vi "Shoot Controller.vi"(8 "error in":errorcluster) -> ()   [LabVIEW 2025]
doc: "This VI executes continuously carrying out the current operation and responding to updates or new operations. It will often contain the timing or control code that is difficult to place directly in TeleOp. This VI generally opens all sensors and motors and isolates the rest of the robot code from knowing how the operations are carried out."
uses:
  <vilib>/Rock Robotics/WPI/Framework/Completion Status.ctl
  <vilib>/Rock Robotics/WPI/ThirdParty/REV Robotics/REVLib/Typedef/SPARK PID Gains.ctl
  <vilib>/Rock Robotics/WPI/ThirdParty/REV Robotics/REVLib/Typedef/SPARK Feed Forward Gains.ctl
  Shoot Setpoints.ctl
  Shoot Operations.ctl
  <vilib>/Rock Robotics/WPI/ThirdParty/REV Robotics/REVLib/Typedef/Spark MAX Control Type.ctl
  79b9af25-1ada-4b96-a7ac-b17063e53c1a.vi
  c9f4092f-8ff2-42f3-87f9-18e20bac81df.vi
  8d211d2e-a7e4-4be3-a004-de462b7f292d.vi
  2d0b4ef1-ddff-4f8f-9f7d-9574eeafe7ac.vi
  <vilib>/Rock Robotics/WPI/ThirdParty/REV Robotics/REVLib/SubVI/Public/SPARK Open Brushless.vi
  <vilib>/Rock Robotics/WPI/ThirdParty/REV Robotics/REVLib/SubVI/Public/SPARK Get Encoder Status Velocity.vi
  <vilib>/Rock Robotics/WPI/ThirdParty/REV Robotics/REVLib/SubVI/Public/SPARK Configure Closed Loop Gains.vi
  <vilib>/Rock Robotics/WPI/ThirdParty/REV Robotics/REVLib/SubVI/Public/SPARK Configure Closed Loop Output Range.vi
  <vilib>/Rock Robotics/Network Tables/NT Write Boolean.vi
panel:
  in  "PID Gains I":T1={"kP"=1e-05, "kI"=0.0, "kD"=0.0}
  in  "Feed Forward Gains I":T2={"kV"=0.003, "kS"=0.0, "kA"=0.0, "kG"=0.0, "kCos"=0.0, "kCosRatio"=0.0}
  in  "Max out Intake":dbl=1.0
  in  "Min out Intake":dbl=-1.0
  out "Intake":T3(graph)
  out "Shooter":T3(graph)
  in  "Intake/Agitater speed":dbl=2500.0
  in  "Shooter Speed":dbl=-5676.0
  in  "Max out Shooter":dbl=1.0
  in  "Min out Shooter":dbl=-1.0
  in  "Feed Forward Gains S":T2={"kV"=0.0021, "kS"=0.0, "kA"=0.0, "kG"=0.0, "kCos"=0.0, "kCosRatio"=0.0}
  in  "PID Gains S":T1={"kP"=0.0001, "kI"=0.0, "kD"=0.0}
  out "Current\nCmd":string="Started at  23:18:34.977\n: Immediate,  S 0.0, D 0.000000"
  in  "Buttons":cluster{"Execute Cmd":bool, "Abort Cmd":bool}
  out "Command Timing":cluster{"Start Time (ms)":u32, "Iterations":i32}
  out "Status":T4
  # "Interactive Command: You may fill in the settings for a command\nand schedule it with the Execute button. You can observe and abort\nany command while fine tuning the code for the controller."
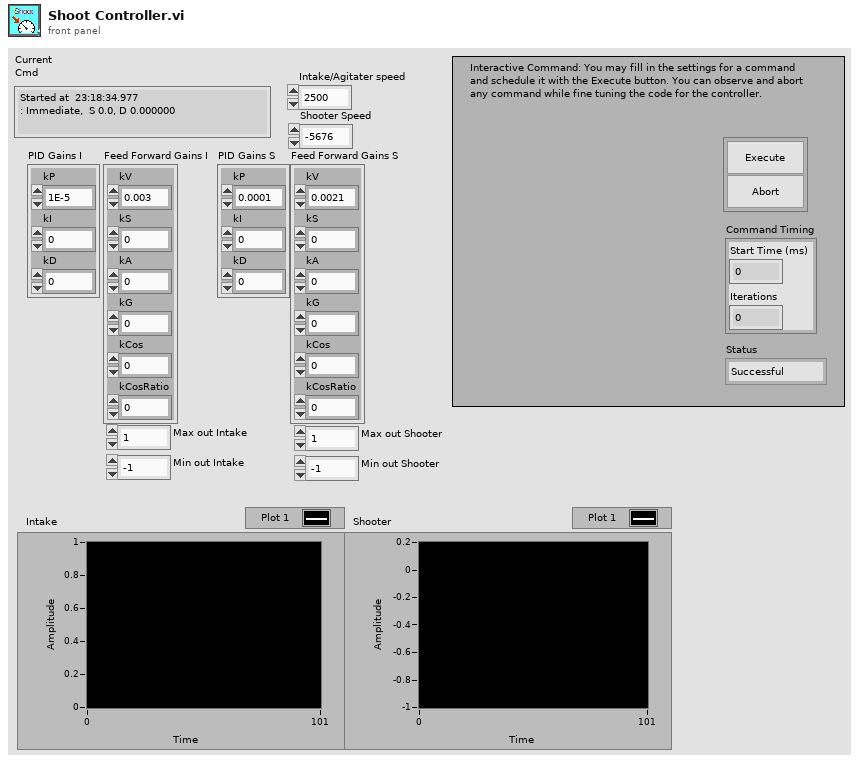
[diagram p1: front panel]
types:
  T1 = typedef "SPARK PID Gains.ctl" = cluster{"kP":dbl, "kI":dbl, "kD":dbl}
  T2 = typedef "SPARK Feed Forward Gains.ctl" = cluster{"kV":dbl, "kS":dbl, "kA":dbl, "kG":dbl, "kCos":dbl, "kCosRatio":dbl}
  T3 = cluster{"Don't move motors while reserved":dbl, "Sensor Velocity":dbl}
  T4 = typedef "Completion Status.ctl" = enum16{"Successful", "Aborted", "Incomplete"}
  T5 = typedef "Shoot Setpoints.ctl" = cluster{"Operation":T6, "Invert Intake":bool, "Shoot":bool, "Intake":bool}
  T6 = typedef "Shoot Operations.ctl" = enum16{"Reserve", "Read Current", "Immediate", "Shoot fuel out the top, intake, and agitate the fuel."}
  T7 = typedef "Command Status Info.ctl" = cluster{"Name":string, "Status":T4, "notifier out":T8}
  T8 = typedef "Completion Notifier.ctl" = refnum<notifier>
  T9 = cluster{"Current Command":T5, "Command Timing":cluster{"Start Time (ms)":u32, "Iterations":i32}, "Command Arguments":cluster{"Command Info":T7, "Description":string, "Default Command":T5, "queue out":refnum<queue>, "Subsystem Name":string}}
  T10 = typedef "WPI_MotorControlDeviceRef.ctl" = cluster{"DeviceStatus":errorcluster, "Type":T11, "PWM":cluster{"PWM Channel":T12, "DeadBand":T13}, "CAN":cluster{"Device Number":u8, "SetOutput VI Ref":variant, "GetOutput VI Ref":variant, "Enable VI Ref":variant, "Disable VI Ref":variant, "Data":variant}, "Invert":bool, "DIO PWM":cluster{"PWM \"Enable\" Channel":T12, "DIOChannel":T14, "PWM Rate":dbl}}
  T11 = typedef "WPI_MotorControlType.ctl" = enum16{"PWM", "CAN", "DIO PWM"}
  T12 = typedef "FPGA_DIOPWMChannel.ctl" = enum8{"PWM 0", "PWM 1", "PWM 2", "PWM 3", "PWM 4", "PWM 5", "PWM 6", "PWM 7", "PWM 8", "PWM 9", "PWM MXP 0", "PWM MXP 1", "PWM MXP 2", "PWM MXP 3", "PWM MXP 4", "PWM MXP 5", "PWM MXP 6", "PWM MXP 7", "PWM MXP 8", "PWM MXP 9", "Invalid"}
  T13 = typedef "WPI_PWMDeadband.ctl" = cluster{"Name":string, "maxPositivePwm":i32, "minPositivePwm":i32, "centerPwm":i32, "maxNegativePwm":i32, "minNegativePwm":i32, "angularRange":u16}
  T14 = typedef "FPGA_DIOChannel.ctl" = enum8{"DIO 0", "DIO 1", "DIO 2", "DIO 3", "DIO 4", "DIO 5", "DIO 6", "DIO 7", "DIO 8", "DIO 9", "DIO MXP 0", "DIO MXP 1", "DIO MXP 2", "DIO MXP 3", "DIO MXP 4", "DIO MXP 5", "DIO MXP 6", "DIO MXP 7", "DIO MXP 8", "DIO MXP 9", "DIO MXP 10", "DIO MXP 11", "DIO MXP 12", "DIO MXP 13", "DIO MXP 14", "DIO MXP 15", "SPI Port CS1", "SPI Port CS2", "SPI Port CS3", "SPI Port MISO", "SPI Port MOSI", "Invalid"}
  T15 = cluster{"Min out Intake":dbl, "Sensor Velocity":dbl}
  T16 = cluster{"Max out Intake":dbl, "Sensor Velocity":dbl}
  T17 = typedef "Spark MAX Control Type.ctl" = enum16{"Percent VBus", "Voltage", "Velocity", "Position", "Smart Motion", "Current", "Smart Velocity", "MAXMotion Position", "MAXMotion Velocity"}
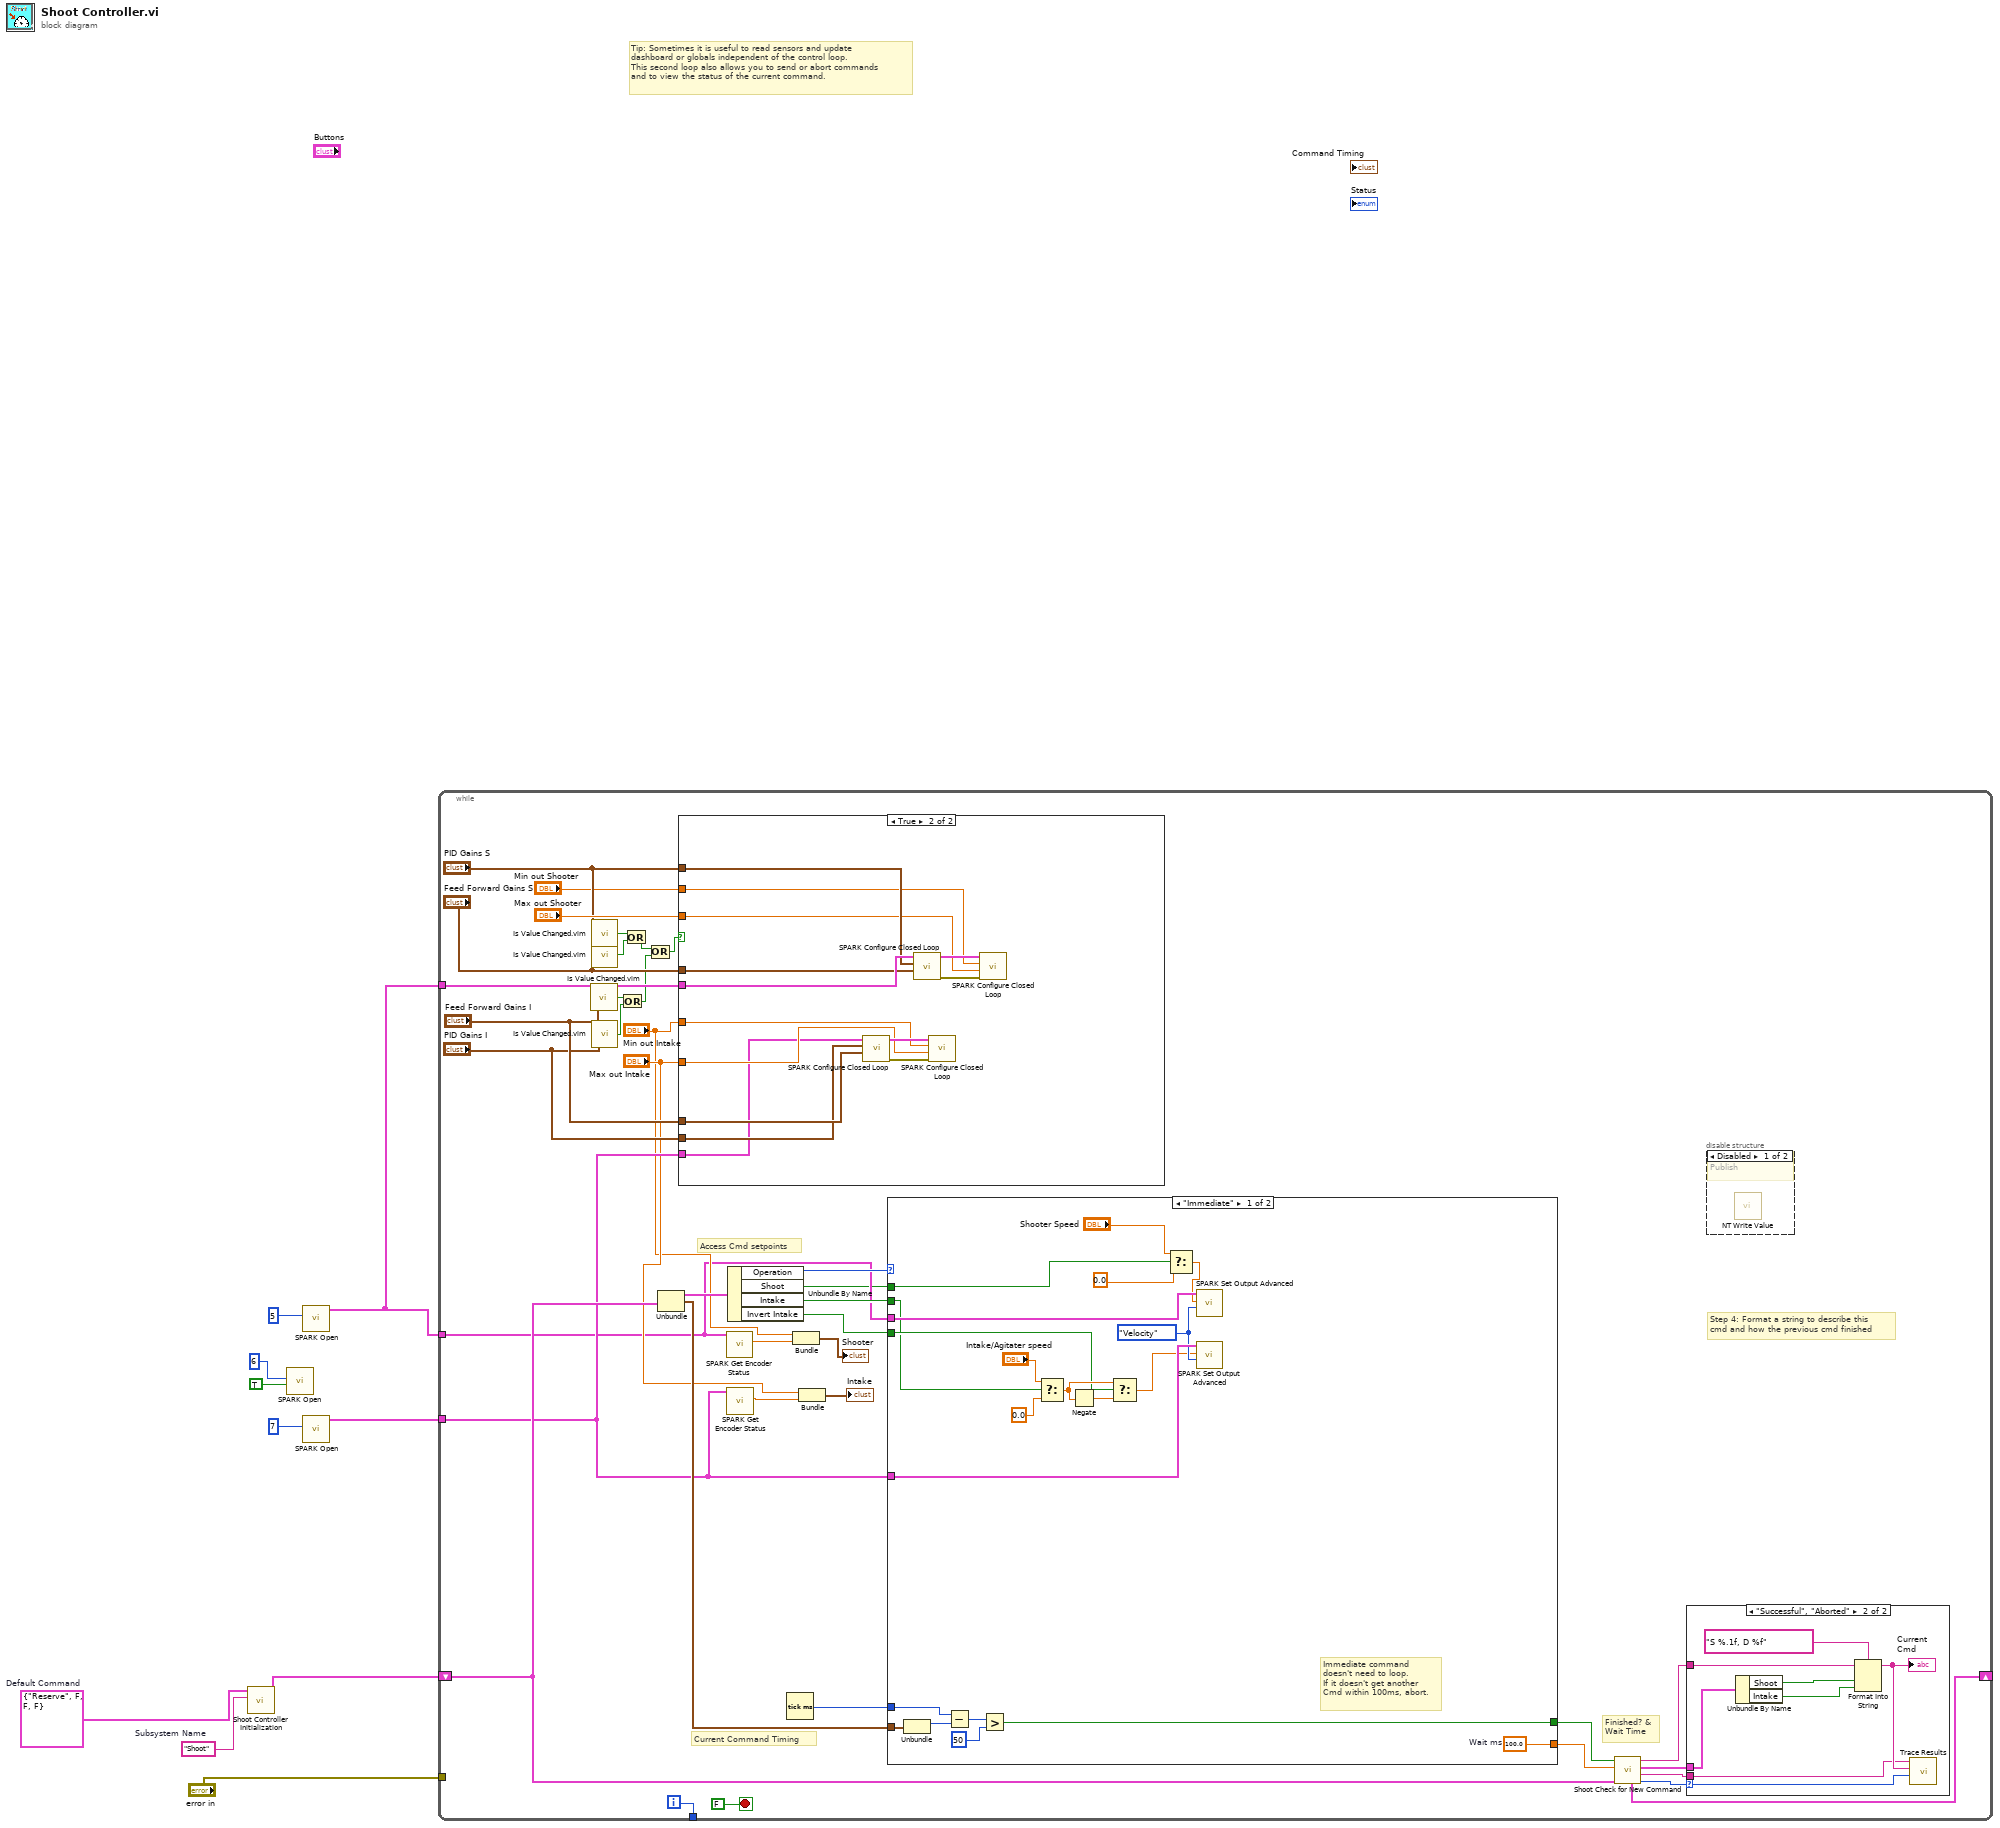
[diagram p0: block diagram]
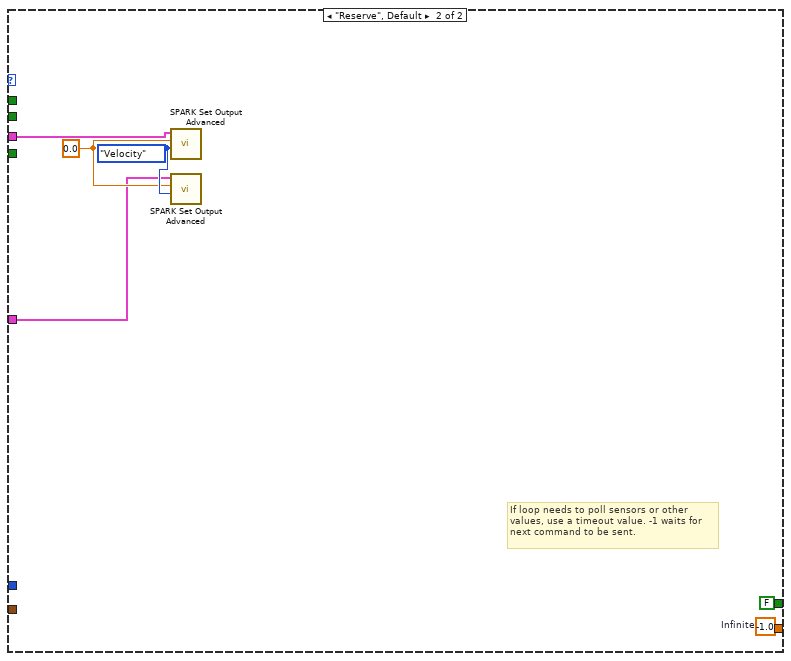
[diagram p5: hidden frame]
diagram:
  w7 = T5 {"Operation"=enum."Reserve", "Invert Intake"=FALSE, "Shoot"=FALSE, "Intake"=FALSE}  # Default Command
  w8 = "Shoot"  # Subsystem Name
  # "Tip: Sometimes it is useful to read sensors and update\ndashboard or globals independent of the control loop.\nThis second loop also allows you to send or abort commands\nand to view the status of the current command."
  n1 = call "Shoot Controller Initialization.vi"("Subsystem Name"=w8, "Default Command"=w7) -> ("Current Command"=w9:T9)  [unwired: 9 in]
  n2 = call-poly <vilib>:"SPARK Open.vi"("Invert"=TRUE, "Device Number"=u8 6) -> ()  [unwired: 8 in, 2 out]
  n3 = call-poly <vilib>:"SPARK Open.vi"("Device Number"=u8 5) -> ("MotorControlDeviceRef"=w1:T10)  [unwired: 9 in, 1 out]
  n4 = call-poly <vilib>:"SPARK Open.vi"("Device Number"=u8 7) -> ("MotorControlDeviceRef"=w3:T10)  [unwired: 9 in, 1 out]
  n5 = while {
    shift-right: [w43] -> _
    shift-left: w9 -> [w36]
    tunnel: [w48] -> _
    tunnel: "error in" -> [_]
    tunnel: w1 -> [w35]
    tunnel: w3 -> [w18]
    tunnel: w1 -> [w13]
    i -> [w48]
    stop <- FALSE stop-if-true
    # "Step 4: Format a string to describe this\ncmd and how the previous cmd finished"
    # "Current Command Timing"
    # "Access Cmd setpoints"
    # "Finished? &\nWait Time"
    n6 = call "Is Value Changed.vim"("value"="Feed Forward Gains I") -> ("changed or first call?"=w24:bool)
    n7 = call "Is Value Changed.vim"("value"="PID Gains S") -> ("changed or first call?"=w34:bool)
    n8 = call "Is Value Changed.vim"("value"="Feed Forward Gains S") -> ("changed or first call?"=w30:bool)
    n9 = call "Is Value Changed.vim"("value"="PID Gains I") -> ("changed or first call?"=w25:bool)
    n10 = Or(x=w24, y=w25) -> (x .or. y?=w26:bool)
    n11 = Or(x=w34, y=w30) -> (x .or. y?=w27:bool)
    n12 = Or(x=w27, y=w26) -> (x .or. y?=w12:bool)
    n13 = Unbundle(w36) -> ("Current Command"=w47:T5, "Command Timing"=w44:cluster{"Start Time (ms)":u32, "Iterations":i32})  [unwired: 1 out]
    n14 = case shown="True" w12 {
      tunnel: w35 -> [_ w63]
      tunnel: "PID Gains S" -> [_ w60]
      tunnel: "Feed Forward Gains S" -> [_ w59]
      tunnel: "Min out Shooter" -> [_ w58]
      tunnel: "Max out Shooter" -> [_ w57]
      tunnel: "Min out Intake" -> [_ w53]
      tunnel: "Max out Intake" -> [_ w54]
      tunnel: "Feed Forward Gains I" -> [_ w52]
      tunnel: "PID Gains I" -> [_ w51]
      tunnel: w18 -> [_ w50]
      frame False {
      }
      frame True {
        n15 = call-poly <vilib>:"SPARK Configure Closed Loop.vi"("Feed Forward Gains"=w52, "PID Gains"=w51, "MotorControlDeviceRef in"=w50) -> ("error out"=w55:errorcluster, "MotorControlDeviceRef out"=w56:T10)  [unwired: 7 in]
        n16 = call-poly <vilib>:"SPARK Configure Closed Loop.vi"("Feed Forward Gains"=w59, "PID Gains"=w60, "MotorControlDeviceRef in"=w63) -> ("error out"=w61:errorcluster, "MotorControlDeviceRef out"=w62:T10)  [unwired: 7 in]
        n17 = call-poly <vilib>:"SPARK Configure Closed Loop.vi"("error in"=w55, "Maximum Output"=w54, "Minimum Output"=w53, "MotorControlDeviceRef in"=w56) -> ()  [unwired: 6 in, 2 out]
        n18 = call-poly <vilib>:"SPARK Configure Closed Loop.vi"("error in"=w61, "Maximum Output"=w57, "Minimum Output"=w58, "MotorControlDeviceRef in"=w62) -> ()  [unwired: 6 in, 2 out]
      }
    }
    n19 = call-poly <vilib>:"SPARK Get Encoder Status.vi"("MotorControlDevRef in"=w13) -> ("Sensor Velocity"=w19:dbl)  [unwired: 7 in, 3 out]
    n20 = call-poly <vilib>:"SPARK Get Encoder Status.vi"("MotorControlDevRef in"=w18) -> ("Sensor Velocity"=w21:dbl)  [unwired: 7 in, 3 out]
    n21 = Unbundle By Name(w47) -> ("Operation"=w46:T6, "Shoot"=w11:bool, "Intake"=w20:bool, "Invert Intake"=w28:bool)
    n22 = Tick Count (ms)() -> (millisecond timer value=w45:u32)
    n23 = Bundle("Min out Intake"="Min out Intake", "Sensor Velocity"=w19) -> (→"Shooter":T15)  [unwired: 1 in]
    n24 = Bundle("Max out Intake"="Max out Intake", "Sensor Velocity"=w21) -> (→"Intake":T16)  [unwired: 1 in]
    n25 = case shown="\"Immediate\"" w46 {
      tunnel: [w92 w98] -> w41
      tunnel: [w86 FALSE ("ignore previous (F)")] -> w42
      tunnel: w44 -> [w88 _]
      tunnel: w11 -> [w72 _]
      tunnel: w45 -> [w87 _]
      tunnel: w20 -> [w73 _]
      tunnel: w13 -> [w85 w96]
      tunnel: w18 -> [w84 w93]
      tunnel: w28 -> [w76 _]
      frame "Immediate" {
        w83 = Spark_MAX_Control_Type."Velocity" ("Control Mode")
        w92 = 100.0  # Wait ms
        # "Immediate command\ndoesn't need to loop.\nIf it doesn't get another\nCmd within 100ms, abort."
        n26 = Unbundle(w88) -> ("Start Time (ms)"=w91:u32)  [unwired: 1 out]
        n27 = Subtract(x=w87, y=w91) -> (x-y=w90:u32)
        n28 = Greater?(x=w90, y=u8 50 ("Left Motor")) -> (0:w86:bool)
        n29 = Select(t="Intake/Agitater speed", s=w73, f=0.0) -> (s? t:f=w77:dbl)
        n30 = Negate(x=w77) -> (-x=w78:dbl)
        n31 = Select(t=w77, s=w76, f=w78) -> (s? t:f=w74:dbl)
        n32 = Select(t="Shooter Speed", s=w72, f=0.0) -> (s? t:f=w75:dbl)
        n33 = call <vilib>:"SPARK Set Output Advanced.vi"("Control Mode"=w83, "Setpoint"=w75, "MotorControlDevRef"=w85) -> ()  [unwired: 7 in, 2 out]
        n34 = call <vilib>:"SPARK Set Output Advanced.vi"("Control Mode"=w83, "Setpoint"=w74, "MotorControlDevRef"=w84) -> ()  [unwired: 7 in, 2 out]
      }
      frame "Reserve", Default {
        w94 = 0.0 ("Setpoint")
        w95 = Spark_MAX_Control_Type."Velocity" ("Control Mode")
        w98 = -1.0  # Infinite
        # "If loop needs to poll sensors or other\nvalues, use a timeout value. -1 waits for\nnext command to be sent."
        n35 = call <vilib>:"SPARK Set Output Advanced.vi"("Control Mode"=w95, "Setpoint"=w94, "MotorControlDevRef"=w96) -> ()  [unwired: 7 in, 2 out]
        n36 = call <vilib>:"SPARK Set Output Advanced.vi"("Control Mode"=w95, "Setpoint"=w94, "MotorControlDevRef"=w93) -> ()  [unwired: 7 in, 2 out]
      }
    }
    n37 = call "Shoot Check for New Command.vi"("Current Command"=w36, "Wait time (ms)"=w41, "Finished?"=w42) -> ("Completion"=w37:T4, "Subsystem Name"=w38:string, "Current Command"=w39:T5, "Initial Trace String"=w40:string, "NextCommand"=w43:T9)  [unwired: 4 in]
    n38 = case shown="\"Successful\", \"Aborted\"" w37 {
      selector: w37 -> [_ w71]
      tunnel: w40 -> [_ w67]
      tunnel: w39 -> [_ w68]
      tunnel: w38 -> [_ w64]
      frame "Incomplete", Default {
        # "Continuing current command"
      }
      frame "Successful", "Aborted" {
        # "Report and setup for next command"
        n39 = Unbundle By Name(w68) -> ("Shoot"=w70:bool, "Intake"=w65:bool)
        n40 = Format Into String(format string="S %.1f, D %f", initial string=w67, w70, w65) -> (resulting string=w66:string)  [unwired: 1 in, 1 out]
        "Current\nCmd" <- w66
        n41 = call <vilib>:"Trace Results.vi"("Status of previous command"=w71, "Description"=w66, "Subsystem"=w64) -> ()  [unwired: 9 in]
      }
    }
    n42 = disable-structure shown="Disabled" {
      frame Disabled {
        # "Publish"
        n43 = call-poly <vilib>:"NT Write Value.vi"() -> ()  [unwired: 11 in, 1 out]
      }
      frame Enabled {
      }
    }
  }
